vi "Test_Echo_Classify.vi"() -> ()   [LabVIEW 2021]
uses:
  C_RX_Buffers.ctl
  CANsub_C.lvlib
  echo/Echo_Context.ctl
  echo/Echo_Frame_Kind.ctl
  echo/Echo_Frame.ctl
panel:
  out "error out":errorcluster
  out "frames":T1[](array[typedef]) {"id" format="%.0x"}
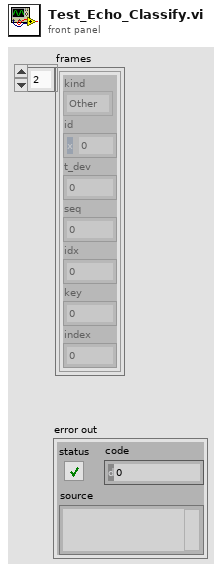
[diagram p1: front panel]
types:
  T1 = typedef "Echo_Frame.ctl" = cluster{"kind":T2, "id":u32, "t_dev":dbl, "seq":u16, "idx":u8, "key":i32, "index":i32}
  T2 = typedef "Echo_Frame_Kind.ctl" = enum16{"Other", "Test", "Ack"}
  T3 = typedef "Echo_Context.ctl" = cluster{"TLS connection":refnum<k5>, "udp":refnum<k16>, "lv addr":u32, "report port":u16, "test lo":u32, "test hi":u32, "ack lo":u32, "ack hi":u32, "echo offset":i32}
  T4 = typedef "CANsub_C.lvlib/C_RX_Buffers.ctl" = cluster{"t_dev":dbl[], "ws":u8[], "id":u32[], "flags":u16[], "hdlc":u8[], "dlc":u8[], "data len":u8[], "data":u8[], "ping":u8[]}
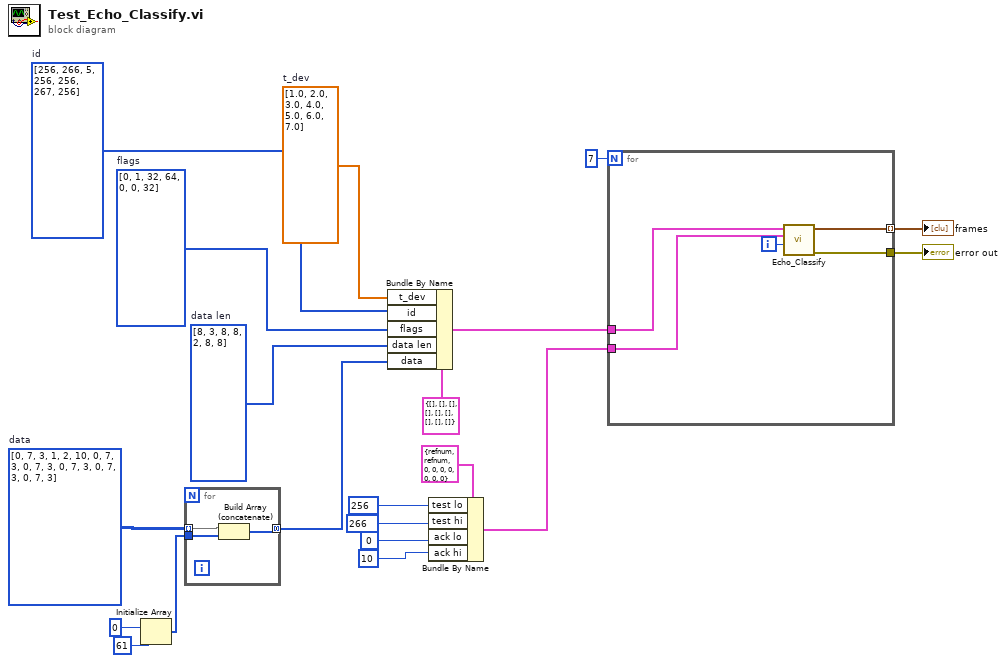
[diagram p0: block diagram]
diagram:
  w19 = u8[][] [[0, 7, 3], [1, 2, 10], [0, 7, 3], [0, 7, 3], [0, 7, 3], [0, 7, 3], [0, 7, 3]]  # data
  w17 = dbl[] [1.0, 2.0, 3.0, 4.0, 5.0, 6.0, 7.0]  # t_dev
  w14 = u8[] [8, 3, 8, 8, 2, 8, 8]  # data len
  w15 = u16[] [0, 1, 32, 64, 0, 0, 32]  # flags
  w16 = u32[] [256, 266, 5, 256, 256, 267, 256]  # id
  n1 = Initialize Array(u8 0, 61 ("dimension size")) -> (w1:u8[])
  n2 = for {
    tunnel: w19 -> [w23] mode=indexing
    tunnel: [w22] -> w18 mode=concatenating
    tunnel: w1 -> [w21]
    n3 = Build Array (concatenate)(w23, w21) -> (w22:u8[])
  }
  n4 = Bundle By Name(cluster=T4 {"t_dev"=[], "ws"=[], "id"=[], "flags"=[], "hdlc"=[], "dlc"=[], "data len"=[], "data"=[], "ping"=[]} ("C_RX_Buffers"), "t_dev"=w17, "id"=w16, "flags"=w15, "data len"=w14, "data"=w18) -> (w7:T4)
  n5 = Bundle By Name(cluster=T3 {"TLS connection"=refnum, "udp"=refnum, "lv addr"=0, "report port"=0, "test lo"=0, "test hi"=0, "ack lo"=0, "ack hi"=0, "echo offset"=0} ("Echo_Context"), "test lo"=u32 256, "test hi"=u32 266 ("test lo"), "ack lo"=u32 0 ("test lo"), "ack hi"=u32 10 ("test lo")) -> (w6:T3)
  n6 = for {
    N: 7 -> [_]
    tunnel: w7 -> [w26]
    tunnel: w6 -> [w25]
    tunnel: [w27] -> w5 mode=indexing
    tunnel: [w24] -> w4
    i -> [w28]
    n7 = call "Echo_Classify.vi"("i"=w28, "context"=w25, "buffers"=w26) -> ("error out"=w24:errorcluster, "frame"=w27:T1)  [unwired: 7 in]
  }
  "frames" <- w5
  "error out" <- w4
